vi "measure 6GHz OOB Measurement.vi"(8 "error in (no error)":errorcluster, 10 "Center Freq(MHz)":dbl, 11 "SA Measurement in":refnum<class "SA Measurement.lvclass">) -> (0 "error out":errorcluster, 2 "Pass?":bool, 3 "SA Measurement out":refnum<class "SA Measurement.lvclass">)   [LabVIEW 2023, in "Spectrum Analyzer.lvlib" / "SA Measurement.lvclass"]
uses:
  SA Measurement.lvclass
  SA Measurement.lvclass/SA Measurement.ctl
  TYPE DEFINITION/Keysight 9020A/TYPE Measurement Preset.ctl
  Spectrum Analyzer.lvlib
  TYPE DEFINITION/TYPE RBW and VBW Select.ctl
  Interface_Spectrum/Interface_Spectrum.lvclass
  TYPE DEFINITION/TYPE Limit Line Setting Table.ctl
  TYPE DEFINITION/TYPE Marker Peak Search Type.ctl
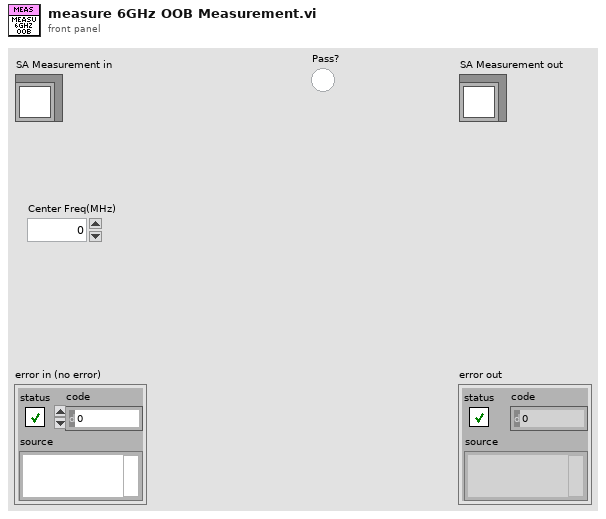
[diagram p1: front panel]
types:
  T1 = typedef "Spectrum Analyzer.lvlib/TYPE Marker Peak Search Type.ctl" = enum16{"Max", "Next Peak"}
  T2 = typedef "Spectrum Analyzer.lvlib/TYPE Limit Line Setting Table.ctl" = cluster{"Limit Line Index":i32, "Frequency Table":dbl[], "Amplitude Table":dbl[], "Name":string}
  T3 = typedef "Spectrum Analyzer.lvlib/TYPE RBW and VBW Select.ctl" = enum16{"Res BW", "Video BW"}
  T4 = typedef "Spectrum Analyzer.lvlib/TYPE Measurement Preset.ctl" = enum16{"Sweep SA Mode", "Channel Power", "Occupied BW", "ACP", "Spurious Emission", "Spurious Emission Mask", "Burst Power (Transmit Power)"}
  T5 = typedef "Spectrum Analyzer.lvlib/TYPE Mask Table for SEM.ctl" = map{enum16{"-10dBm Upper", "-10dBm Lower"}, map{dbl, map{i32, cluster{"Freq":dbl, "Limit":dbl, "dBc Applied?":bool}[]}}}
  T6 = typedef "Spectrum Analyzer.lvlib/TYPE Y-axis Unit.ctl" = enum16{"dBm", "dBmV", "dBuV", "dBpW", "Volt", "Ampere", "Watt"}
  T7 = typedef "Spectrum Analyzer.lvlib/TYPE Reference Level and Atten Param.ctl" = cluster{"Reference Level":dbl, "Atten":i32, "Atten Auto?":bool, "Reference Level Offset":dbl}
  T8 = typedef "Spectrum Analyzer.lvlib/TYPE Start and Stop Frequency.ctl" = cluster{"Start":dbl, "Stop":dbl}
  T9 = typedef "Spectrum Analyzer.lvlib/TYPE Display Trace Mode Select.ctl" = enum16{"Clear Write", "Max Hold", "Min Hold", "Average", "View"}
  T10 = typedef "Spectrum Analyzer.lvlib/TYPE Detect Mode Select.ctl" = enum16{"Det Auto (Normal)", "Auto Peak", "Positive Peak", "Negative Peak", "Sample", "RMS", "Average", "Quasipeak", "CISPR Average", "RMS Average"}
  T11 = cluster{"Trace Mode":T9, "Detector Type":T10, "Detect Auto?":bool}[]
  T12 = typedef "Spectrum Analyzer.lvlib/TYPE Average Mode Select.ctl" = enum16{"Linear(Voltage Avg)", "Video(Log)", "Power"}
  T13 = typedef "Spectrum Analyzer.lvlib/TYPE Marker Value.ctl" = cluster{"X-axis":dbl, "Y-axis":dbl}
  T14 = map{dbl, map{i32, cluster{"Freq":dbl, "Limit":dbl, "dBc Applied?":bool}[]}}
  T15 = map{i32, cluster{"Freq":dbl, "Limit":dbl, "dBc Applied?":bool}[]}
  T16 = cluster{"Freq":dbl, "Limit":dbl, "dBc Applied?":bool}[]
  T17 = typedef "Spectrum Analyzer.lvlib/TYPE Trace Value Array.ctl" = cluster{"Frequency":dbl[], "Amplitude":dbl[]}
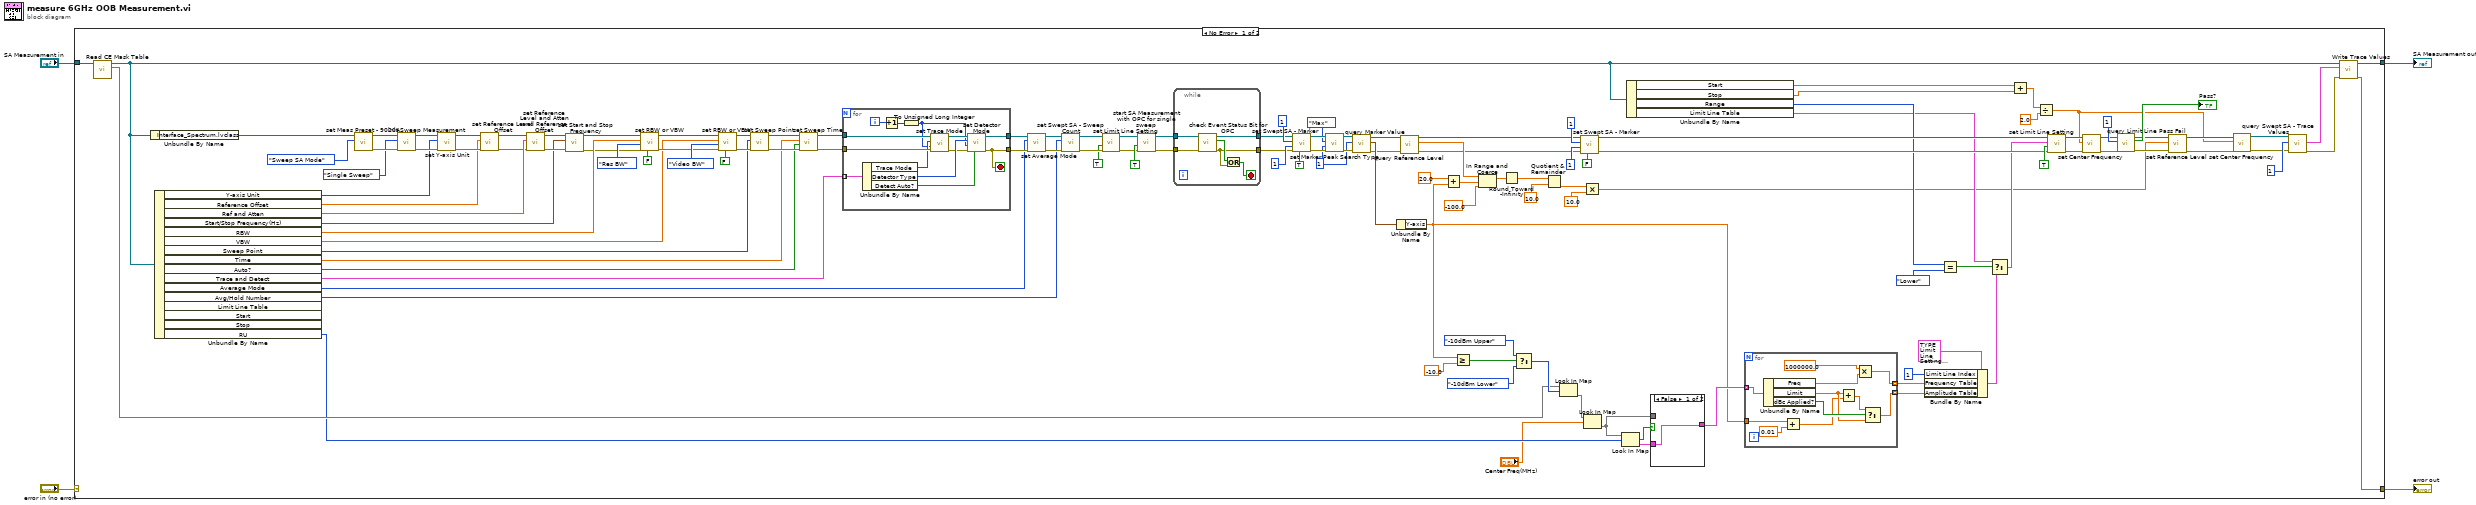
[diagram p0: block diagram]
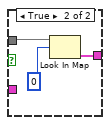
[diagram p2: hidden frame]
diagram:
  n1 = case shown="No Error" "error in (no error)" {
    selector: "error in (no error)" -> [_ w171]
    tunnel: [w16 w171] -> w1
    tunnel: [w17 w170] -> w2
    tunnel: "SA Measurement in" -> [w88 w170]
    frame No Error {
      w69 = 1 ("Marker Index")
      n2 = call "Read CE Mask Table.vi"("SA Measurement in"=w88) -> ("Mask Table"=w50:T5, "SA Measurement out"=w15:refnum<class "SA Measurement.lvclass">)  [unwired: 8 in, 1 out]
      n3 = Unbundle By Name(w15) -> ("Interface_Spectrum.lvclass"=w135:refnum<class "Interface_Spectrum.lvclass">)
      n4 = Unbundle By Name(w15) -> ("Y-axis Unit"=w119:T6, "Reference Offset"=w5:dbl, "Ref and Atten"=w130:T7, "Start/Stop Frequency(Hz)"=w97:T8, "RBW"=w129:dbl, "VBW"=w122:dbl, "Sweep Point"=w116:u32, "Time"=w113:dbl, "Auto?"=w112:bool, "Trace and Detect"=w109:T11, "Average Mode"=w106:T12, "Avg/Hold Number"=w103:u32, "RU"=w45:i32)  [unwired: 3 out]
      n5 = call-dynamic "set Meas Preset - 9020A.vi"("Measurement Preset"=TYPE_Measurement_Preset."Sweep SA Mode", "Interface_Spectrum in"=w135) -> ("error out"=w132:errorcluster, "Interface_Spectrum out"=w133:refnum<class "Interface_Spectrum.lvclass">)  [unwired: 8 in]
      n6 = call-dynamic "init Sweep Measurement.vi"("error in (no error)"=w132, "Sweep Measurement Mode"=enum16{"Single Sweep", "Continuous Sweep"}."Single Sweep", "Interface_Spectrum in"=w133) -> ("error out"=w120:errorcluster, "Interface_Spectrum out"=w121:refnum<class "Interface_Spectrum.lvclass">)  [unwired: 7 in]
      n7 = call-dynamic "set Y-axis Unit.vi"("error in (no error)"=w120, "Y-axis Unit"=w119, "Interface_Spectrum in"=w121) -> ("error out"=w8:errorcluster, "Interface_Spectrum out"=w9:refnum<class "Interface_Spectrum.lvclass">)  [unwired: 7 in]
      n8 = call-dynamic "set Reference Level Offset.vi"("error in (no error)"=w8, "Reference Level Offset"=w5, "Interface_Spectrum in"=w9) -> ("error out"=w6:errorcluster, "Interface_Spectrum out"=w7:refnum<class "Interface_Spectrum.lvclass">)  [unwired: 7 in]
      n9 = call-dynamic "set Reference Level and Atten and Reference Offset.vi"("error in (no error)"=w6, "Reference Level, Atten, Reference Offset"=w130, "Interface_Spectrum in"=w7) -> ("error out"=w98:errorcluster, "Interface_Spectrum out"=w99:refnum<class "Interface_Spectrum.lvclass">)  [unwired: 7 in]
      n10 = call-dynamic "set Start and Stop Frequency.vi"("error in (no error)"=w98, "Start/Stop Frequency(Hz)"=w97, "Interface_Spectrum in"=w99) -> ("error out"=w95:errorcluster, "Interface_Spectrum out"=w96:refnum<class "Interface_Spectrum.lvclass">)  [unwired: 7 in]
      n11 = call-dynamic "set RBW or VBW.vi"("BW Auto?"=FALSE, "error in (no error)"=w95, "BW Type"=TYPE_RBW_and_VBW_Select."Res BW", "BW Value (Hz)"=w129, "Interface_Spectrum in"=w96) -> ("error out"=w123:errorcluster, "Interface_Spectrum out"=w124:refnum<class "Interface_Spectrum.lvclass">)  [unwired: 5 in]
      n12 = call-dynamic "set RBW or VBW.vi"("BW Auto?"=FALSE, "error in (no error)"=w123, "BW Type"=TYPE_RBW_and_VBW_Select."Video BW", "BW Value (Hz)"=w122, "Interface_Spectrum in"=w124) -> ("error out"=w117:errorcluster, "Interface_Spectrum out"=w118:refnum<class "Interface_Spectrum.lvclass">)  [unwired: 5 in]
      n13 = call-dynamic "set Sweep Point.vi"("error in (no error)"=w117, "Sweep Point"=w116, "Interface_Spectrum in"=w118) -> ("error out"=w114:errorcluster, "Interface_Spectrum out"=w115:refnum<class "Interface_Spectrum.lvclass">)  [unwired: 7 in]
      n14 = call-dynamic "set Sweep Time.vi"("error in (no error)"=w114, "Sweep Time Auto?"=w112, "Sweep Time(sec)"=w113, "Interface_Spectrum in"=w115) -> ("error out"=w110:errorcluster, "Interface_Spectrum out"=w111:refnum<class "Interface_Spectrum.lvclass">)  [unwired: 6 in]
      n15 = for {
        tunnel: w111 -> [w168]
        tunnel: w110 -> [w167]
        tunnel: w109 -> [w169] mode=indexing
        tunnel: [w157] -> w107
        tunnel: [w158] -> w108
        i -> [w166]
        stop <- w157 stop-if-true
        n16 = Unbundle By Name(w169) -> ("Trace Mode"=w164:T9, "Detector Type"=w162:T10, "Detect Auto?"=w159:bool)
        n17 = Increment(x=w166) -> (x+1=w165:i32)
        n18 = To Unsigned Long Integer(number=w165) -> (unsigned 32bit integer=w160:u32)
        n19 = call-dynamic "set Trace Mode.vi"("error in (no error)"=w167, "Trace Index"=w160, "Trace Mode"=w164, "Interface_Spectrum in"=w168) -> ("error out"=w161:errorcluster, "Interface_Spectrum out"=w163:refnum<class "Interface_Spectrum.lvclass">)  [unwired: 6 in]
        n20 = call-dynamic "set Detector Mode.vi"("Detect Auto?"=w159, "error in (no error)"=w161, "Trace Index"=w160, "Detector Type"=w162, "Interface_Spectrum in"=w163) -> ("error out"=w157:errorcluster, "Interface_Spectrum out"=w158:refnum<class "Interface_Spectrum.lvclass">)  [unwired: 5 in]
      }
      n21 = call-dynamic "set Average Mode.vi"("error in (no error)"=w107, "Average Mode"=w106, "Interface_Spectrum in"=w108) -> ("error out"=w104:errorcluster, "Interface_Spectrum out"=w105:refnum<class "Interface_Spectrum.lvclass">)  [unwired: 7 in]
      n22 = call-dynamic "set Swept SA - Sweep Count.vi"("error in (no error)"=w104, "Sweep Count"=w103, "Interface_Spectrum in"=w105) -> ("error out"=w93:errorcluster, "Interface_Spectrum out"=w94:refnum<class "Interface_Spectrum.lvclass">)  [unwired: 7 in]
      n23 = call-dynamic "set Limit Line Setting.vi"("error in (no error)"=w93, "Turn On?"=TRUE, "Interface_Spectrum in"=w94) -> ("error out"=w90:errorcluster, "Interface_Spectrum out"=w91:refnum<class "Interface_Spectrum.lvclass">)  [unwired: 7 in]
      n24 = call-dynamic "start SA Measurement with OPC for single sweep.vi"("error in (no error)"=w90, "with OPC?"=TRUE, "Interface_Spectrum in"=w91) -> ("error out"=w100:errorcluster, "Interface_Spectrum out"=w101:refnum<class "Interface_Spectrum.lvclass">)  [unwired: 7 in]
      n25 = while {
        tunnel: w101 -> [w156]
        tunnel: w100 -> [w155]
        tunnel: [w152] -> w67
        tunnel: [w151] -> w68
        stop <- w153 stop-if-true
        n26 = call-dynamic "check Event Status Bit for OPC.vi"("error in (no error)"=w155, "Interface_Spectrum in"=w156) -> ("error out"=w152:errorcluster, "OPC Bit Changed?"=w154:bool, "Interface_Spectrum out"=w151:refnum<class "Interface_Spectrum.lvclass">)  [unwired: 7 in]
        n27 = Or(x=w154, y=w152) -> (x .or. y?=w153:bool)
      }
      n28 = call-dynamic "set Swept SA - Marker.vi"("On?"=TRUE, "error in (no error)"=w67, "trace"=1, "Index"=1, "Interface_Spectrum in"=w68) -> ("error out"=w73:errorcluster, "Interface_Spectrum out"=w74:refnum<class "Interface_Spectrum.lvclass">)  [unwired: 5 in]
      n29 = call-dynamic "set Marker Peak Search Type.vi"("error in (no error)"=w73, "Marker Index"=w69, "Peak Search Type"=TYPE_Marker_Peak_Search_Type."Max", "Interface_Spectrum in"=w74) -> ("error out"=w70:errorcluster, "Interface_Spectrum out"=w71:refnum<class "Interface_Spectrum.lvclass">)  [unwired: 6 in]
      n30 = call-dynamic "query Marker Value.vi"("error in (no error)"=w70, "Marker Index"=w69, "Interface_Spectrum in"=w71) -> ("error out"=w36:errorcluster, "Marker Value"=w66:T13, "Interface_Spectrum out"=w37:refnum<class "Interface_Spectrum.lvclass">)  [unwired: 6 in]
      n31 = Unbundle By Name(w66) -> ("Y-axis"=w32:dbl)
      n32 = call-dynamic "query Reference Level.vi"("error in (no error)"=w36, "Interface_Spectrum in"=w37) -> ("error out"=w28:errorcluster, "Ref Level"=w30:dbl, "Interface_Spectrum out"=w29:refnum<class "Interface_Spectrum.lvclass">)  [unwired: 7 in]
      n33 = Add(x=20.0, y=w32) -> (x+y=w35:dbl)
      n34 = Greater Or Equal?(x=w32, y=-10.0) -> (x >= y?=w82:bool)
      n35 = In Range and Coerce(upper limit=w30, x=w35, lower limit=-100.0) -> (coerced(x)=w33:dbl)  [unwired: 1 out]
      n36 = Round Toward -Infinity(1:w33) -> (0:w14:dbl)
      n37 = Select(t=enum16{"-10dBm Upper", "-10dBm Lower"}."-10dBm Upper" ("key"), s=w82, f=enum16{"-10dBm Upper", "-10dBm Lower"}."-10dBm Lower" ("key")) -> (s? t:f=w79:enum16{"-10dBm Upper", "-10dBm Lower"})
      n38 = Quotient & Remainder(x=w14, y=10.0) -> (floor(x/y)=w12:dbl)  [unwired: 1 out]
      n39 = Look In Map(map=w50, key=w79) -> (value=w78:T14)  [unwired: 1 in, 1 out]
      n40 = call-dynamic "set Swept SA - Marker.vi"("On?"=FALSE, "error in (no error)"=w28, "trace"=1, "Index"=1, "Interface_Spectrum in"=w29) -> ("error out"=w59:errorcluster, "Interface_Spectrum out"=w60:refnum<class "Interface_Spectrum.lvclass">)  [unwired: 5 in]
      n41 = Multiply(x=w12, y=10.0) -> (x*y=w10:dbl)
      n42 = Look In Map(map=w78, key="Center Freq(MHz)") -> (value=w47:T15)  [unwired: 1 in, 1 out]
      n43 = Look In Map(map=w47, key=w45) -> (key not found?=w49:bool, value=w48:T16)  [unwired: 1 in]
      n44 = Unbundle By Name(w15) -> ("Start"=w54:dbl, "Stop"=w53:dbl, "Range"=w44:enum16{"Lower", "Upper"}, "Limit Line Table"=w41:T2)
      n45 = case shown="False" w49 {
        tunnel: w48 -> [w136 _]
        tunnel: w47 -> [_ w139]
        tunnel: [w136 w137] -> w46
        frame False {
        }
        frame True {
          n46 = Look In Map(map=w139, key=0) -> (value=w137:T16)  [unwired: 1 in, 1 out]
        }
      }
      n47 = for {
        tunnel: w46 -> [w150] mode=indexing
        tunnel: [w147] -> w85 mode=indexing
        tunnel: [w145] -> w84 mode=indexing
        tunnel: w32 -> [w142]
        n48 = Unbundle By Name(w150) -> ("Freq"=w149:dbl, "Limit"=w143:dbl, "dBc Applied?"=w146:bool)
        n49 = Add(x=w142, y=0.01) -> (x+y=w141:dbl)
        n50 = Add(x=w143, y=w141) -> (x+y=w144:dbl)
        n51 = Multiply(x=1000000.0, y=w149) -> (x*y=w147:dbl)
        n52 = Select(t=w144, s=w146, f=w143) -> (s? t:f=w145:dbl)
      }
      n53 = Bundle By Name(cluster=T2 {"Limit Line Index"=1, "Frequency Table"=[1000000000.0, 2000000000.0, 3000000000.0], "Amplitude Table"=[-60.0, -50.0, -40.0], "Name"=""} ("Limit Line Setting"), "Limit Line Index"=1, "Frequency Table"=w85, "Amplitude Table"=w84) -> (w40:T2)
      n54 = Equal?(x=w44, y=enum16{"Lower", "Upper"}."Lower") -> (x = y?=w42:bool)
      n55 = Select(t=w41, s=w42, f=w40) -> (s? t:f=w39:T2)
      n56 = Add(x=w54, y=w53) -> (x+y=w52:dbl)
      n57 = Divide(x=w52, y=2.0) -> (x/y=w23:dbl)
      n58 = call-dynamic "set Limit Line Setting.vi"("error in (no error)"=w59, "Turn On?"=TRUE, "Limit Line Setting"=w39, "Interface_Spectrum in"=w60) -> ("error out"=w57:errorcluster, "Interface_Spectrum out"=w58:refnum<class "Interface_Spectrum.lvclass">)  [unwired: 6 in]
      n59 = call-dynamic "set Center Frequency.vi"("error in (no error)"=w57, "Center Frequency (Hz)"=w23, "Interface_Spectrum in"=w58) -> ("error out"=w55:errorcluster, "Interface_Spectrum out"=w56:refnum<class "Interface_Spectrum.lvclass">)  [unwired: 7 in]
      n60 = call-dynamic "query Limit Line Pass Fail.vi"("error in (no error)"=w55, "Limit Line Index"=1, "Interface_Spectrum in"=w56) -> ("error out"=w26:errorcluster, "Pass?"=→"Pass?":bool, "Interface_Spectrum out"=w27:refnum<class "Interface_Spectrum.lvclass">)  [unwired: 6 in]
      n61 = call-dynamic "set Reference Level.vi"("error in (no error)"=w26, "Reference Level"=w10, "Interface_Spectrum in"=w27) -> ("error out"=w24:errorcluster, "Interface_Spectrum out"=w25:refnum<class "Interface_Spectrum.lvclass">)  [unwired: 7 in]
      n62 = call-dynamic "set Center Frequency.vi"("error in (no error)"=w24, "Center Frequency (Hz)"=w23, "Interface_Spectrum in"=w25) -> ("error out"=w18:errorcluster, "Interface_Spectrum out"=w19:refnum<class "Interface_Spectrum.lvclass">)  [unwired: 7 in]
      n63 = call-dynamic "query Swept SA - Trace Values.vi"("error in (no error)"=w18, "Trace Index"=u32 1, "Interface_Spectrum in"=w19) -> ("error out"=w21:errorcluster, "Trace Values"=w20:T17)  [unwired: 6 in, 1 out]
      n64 = call "Write Trace Values.vi"("error in (no error)"=w21, "Trace Values"=w20, "SA Measurement in"=w15) -> ("error out"=w16:errorcluster, "SA Measurement out"=w17:refnum<class "SA Measurement.lvclass">)  [unwired: 7 in]
    }
    frame Error {
    }
  }
  "error out" <- w1
  "SA Measurement out" <- w2
